vi "Delete Group.vi"(5 "Save File":bool=TRUE, 6 "error in (no error)":errorcluster, 8 "Group Name":string, 9 "EasyUserManager in":refnum<class "EasyUserManager.lvclass">) -> (0 "error out":errorcluster, 3 "EasyUserManager out":refnum<class "EasyUserManager.lvclass">)   [LabVIEW 2024, in "EasyUserManager.lvclass"]
doc: "Delete the user group specified by <B>Group Name</B>.\n\nThe boolean input <B>Save File</B> controls whether changes are immediately saved to the users file (Default: True)."
uses:
  EasyUserManager.lvclass
  EasyUserManager.lvclass/EasyUserManager.ctl
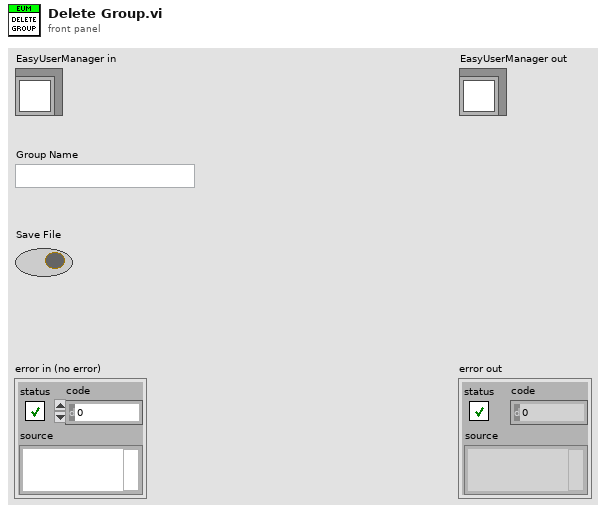
[diagram p1: front panel]
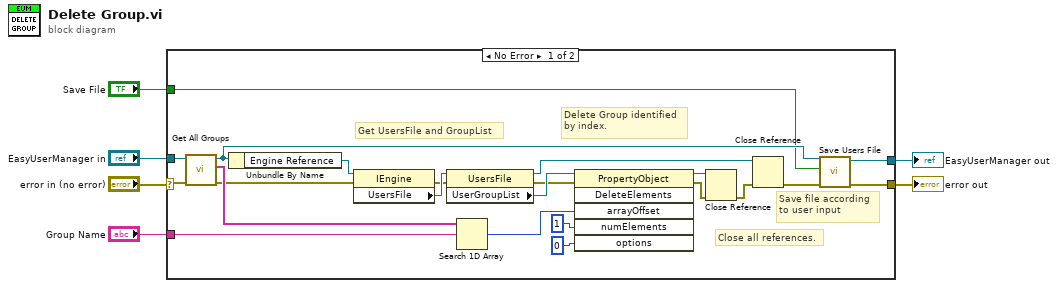
[diagram p0: block diagram]
diagram:
  n1 = case shown="No Error" "error in (no error)" {
    selector: "error in (no error)" -> [w9 w30]
    tunnel: [w24 w30] -> w5
    tunnel: [w25 w29] -> w3
    tunnel: "EasyUserManager in" -> [w28 w29]
    tunnel: "Save File" -> [w8 _]
    tunnel: "Group Name" -> [w7 _]
    frame No Error {
      # "Save file according\nto user input"
      # "Close all references."
      # "Delete Group identified\nby index."
      # "Get UsersFile and GroupList"
      n2 = call "Get All Groups.vi"("error in (no error)"=w9, "EasyUserManager in"=w28) -> ("error out"=w10:errorcluster, "Groups"=w27:string[], "EasyUserManager out"=w26:refnum<class "EasyUserManager.lvclass">)  [unwired: 3 in]
      n3 = Unbundle By Name(w26) -> ("Engine Reference"=w21:refnum<k7>)
      n4 = property on="Property Node" class="IEngine"(reference=w21, error in=w10) -> (error out=w22:errorcluster, "UsersFile"=w23:refnum<k7>)  [unwired: 1 out]
      n5 = property on="Property Node" class="UsersFile"(reference=w23, error in=w22) -> (reference out=w14:refnum<k7>, error out=w16:errorcluster, "UserGroupList"=w18:refnum<k7>)
      n6 = Search 1D Array(1D array=w27, element=w7) -> (index of element=w17:i32)  [unwired: 1 in]
      n7 = invoke on="Invoke Node" class="PropertyObject" method="DeleteElements"(reference=w18, error in=w16, "arrayOffset"=w17, "numElements"=1, "options"=0) -> (reference out=w15:refnum<k7>, error out=w12:errorcluster)  [unwired: 1 in, 4 out]
      n8 = Close Reference(reference=w15, error in (no error)=w12) -> (error out=w13:errorcluster)
      n9 = Close Reference(reference=w14, error in (no error)=w13) -> (error out=w11:errorcluster)
      n10 = call "Save Users File.vi"("error in (no error)"=w11, "Save"=w8, "EasyUserManager in"=w26) -> ("error out"=w24:errorcluster, "EasyUserManager out"=w25:refnum<class "EasyUserManager.lvclass">)  [unwired: 3 in]
    }
    frame Error {
      # "Pass error and do nothing."
    }
  }
  "error out" <- w5
  "EasyUserManager out" <- w3
